vi "get_item_by_name.vi"(8 "error in (no error)":errorcluster, 10 "item_name":string, 11 "Table in":refnum<class "Table.lvclass">) -> (0 "error out":errorcluster, 1 "Item":refnum<class "Item.lvclass">, 2 "found?":bool, 3 "Table out":refnum<class "Table.lvclass">, 5 "item_type":T1)   [LabVIEW 2020, in "toml_edit.lvlib" / "Table.lvclass"]
uses:
  Table.lvclass
  Item/Item.lvclass
  Item/type--enum.ctl
  Table.lvclass/Table.ctl
  dragon_toml_64.dll
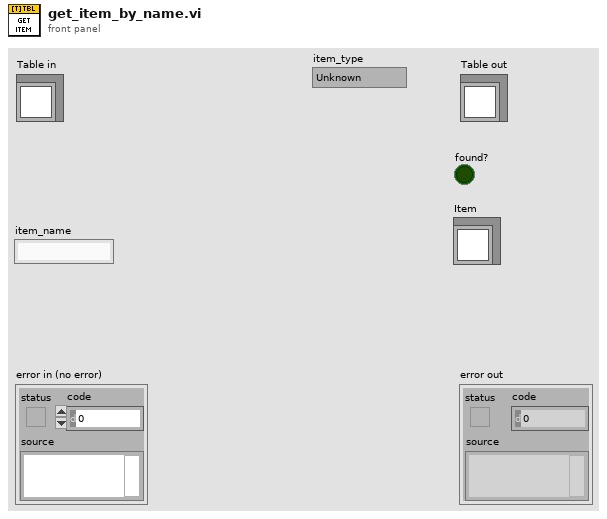
[diagram p1: front panel]
types:
  T1 = typedef "toml_edit.lvlib/Item.lvclass/type--enum.ctl" = enum16{"Unknown", "None", "Value", "ArrayOfTables", "Table"}
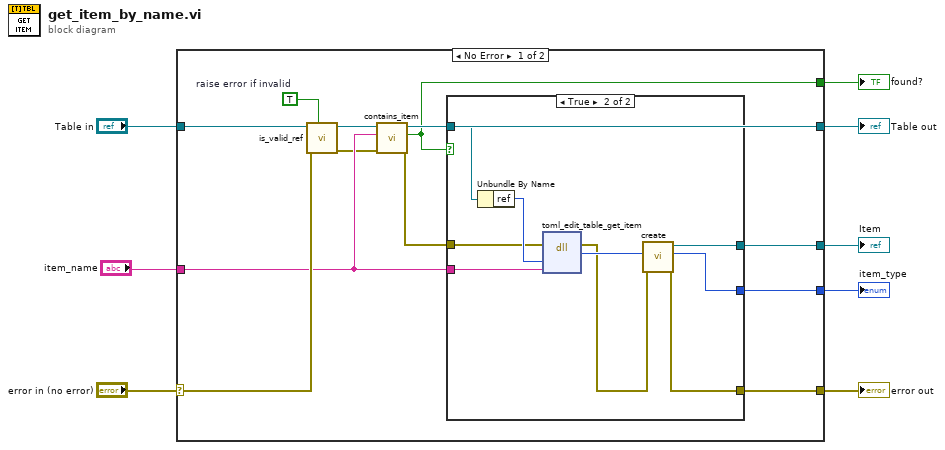
[diagram p0: block diagram]
diagram:
  n1 = case shown="No Error" "error in (no error)" {
    selector: "error in (no error)" -> [w16 w32]
    tunnel: [w19 w32] -> w7
    tunnel: [w13 w31] -> w5
    tunnel: "Table in" -> [w17 w31]
    tunnel: "item_name" -> [w12 _]
    tunnel: [w20 _] -> w3
    tunnel: [w18 _] -> w2
    tunnel: [w9 _] -> w1
    frame No Error {
      w15 = TRUE  # raise error if invalid
      n2 = call-dynamic "is_valid_ref.vi"("raise error if invalid? (False)"=w15, "error in (no error)"=w16, "Table in"=w17) -> ("error out"=w11:errorcluster, "Table out"=w14:refnum<class "Table.lvclass">)  [unwired: 6 in, 1 out]
      n3 = call "contains_item.vi"("error in (no error)"=w11, "item_name"=w12, "Table in"=w14) -> ("error out"=w10:errorcluster, "contains_item"=w9:bool, "Table out"=w13:refnum<class "Table.lvclass">)  [unwired: 6 in]
      n4 = case shown="True" w9 {
        tunnel: [_ w30] -> w20
        tunnel: [w21 w29] -> w19
        tunnel: [_ w28] -> w18
        tunnel: w13 -> [_ w24]
        tunnel: w12 -> [_ w23]
        tunnel: w10 -> [w21 w22]
        frame False {
        }
        frame True {
          n5 = Unbundle By Name(w24) -> ("ref"=w26:u64)
          n6 = dll-call lib="C:/projects/dragon-desktop/source/submodules/toml-edit-labview/lv_src/dragon_toml_*.*" fn="toml_edit_table_get_item"(error in=w22, "table_ref"=w26, "item_name"=w23) -> (error out=w25:errorcluster, "item_ref"=w27:u64)  [unwired: 4 in, 1 out]
          n7 = call "create.vi"("error in (no error)"=w25, "ref"=w27) -> ("error out"=w29:errorcluster, "item_type"=w28:T1, "Item out"=w30:refnum<class "Item.lvclass">)  [unwired: 7 in]
        }
      }
    }
    frame Error {
    }
  }
  "error out" <- w7
  "Table out" <- w5
  "Item" <- w3
  "item_type" <- w2
  "found?" <- w1
